vi "Demo.vi"() -> ()   [LabVIEW 2012]
uses:
  XY Plot with Error Bars.xctl
panel:
  out "Plot:Visible":bool
  in  "XY Plot with Error Bars":cluster{"X":dbl[], "Y":dbl[]}(xcontrol)
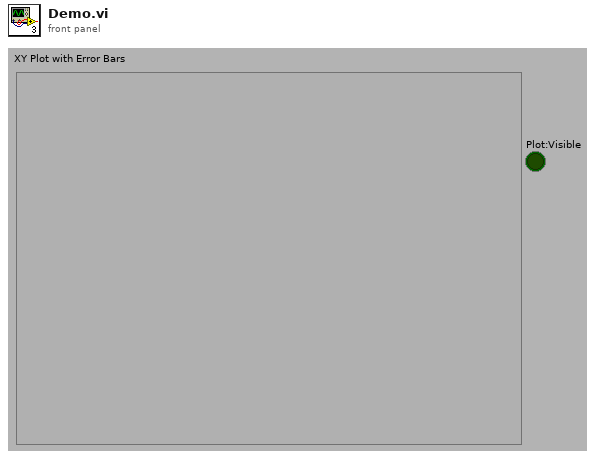
[diagram p1: front panel]
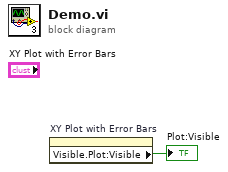
[diagram p0: block diagram]
diagram:
  n1 = property on="XY Plot with Error Bars" class="XY Plot with Error Bars (strict"() -> ("Visible.Plot:Visible"=→"Plot:Visible":bool)  [unwired: 2 in, 2 out]
